vi "Read Name.vi"(8 "error in (no error)":errorcluster, 11 "Process In":refnum<class "Process.lvclass">) -> (0 "error out":errorcluster, 1 "Name":string, 2 "Qualified Name":string, 3 "Process Out":refnum<class "Process.lvclass">)   [LabVIEW 2020, in "Process.lvclass"]
doc: "Returns the name of the object. The Qualified Name is prepended with the name of the owner recursively in the format \"Owner Name::Name\"."
uses:
  Process.lvclass
  C:/git/astemes-triarc-framework/source/Framework/Base/Base.lvclass
  Process.lvclass/Process.ctl
  Base/Base.lvclass/Base.ctl
  <vilib>/Utility/error.llb/Clear Errors.vi
  <vilib>/Utility/error.llb/Error Cluster From Error Code.vi
  Base/Base.lvclass
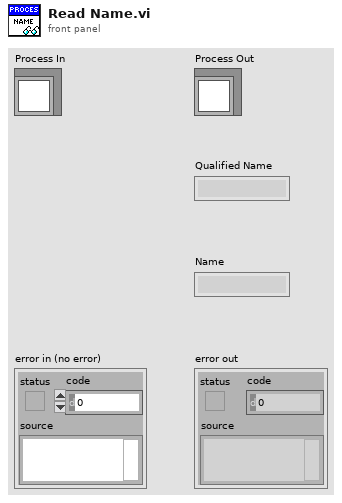
[diagram p1: front panel]
types:
  T1 = typedef "Process.lvclass/Lifecycle State.ctl" = enum16{"Uninitialized", "Initialized", "Started", "Running", "Stopped", "Finished"}
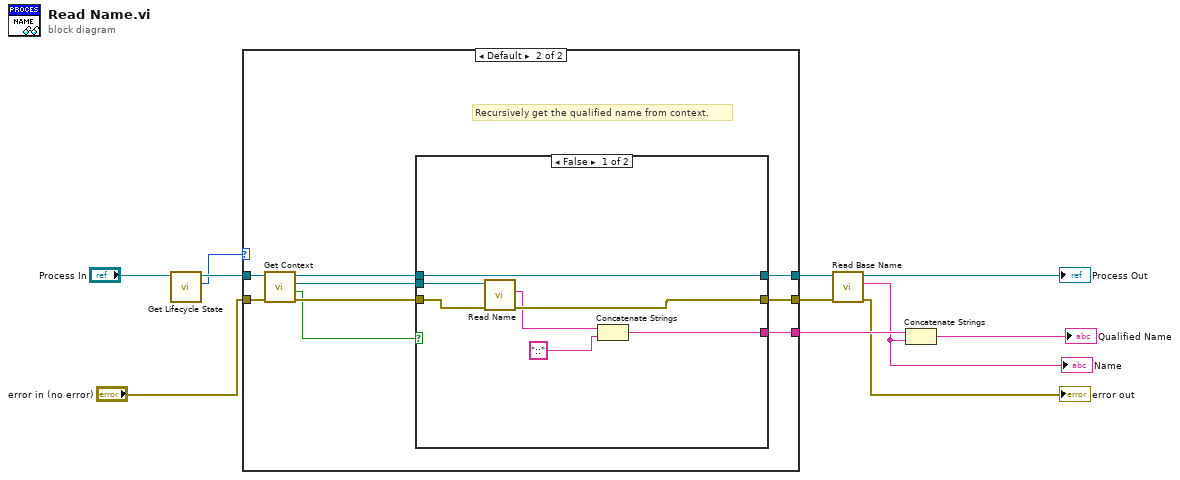
[diagram p0: block diagram]
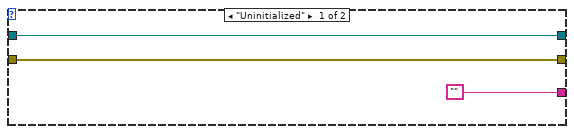
[diagram p2: hidden frame]
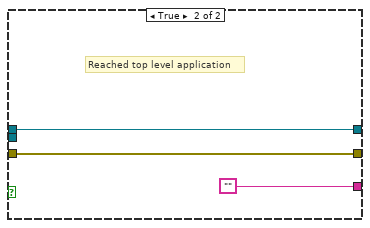
[diagram p3: hidden frame]
diagram:
  n1 = call "Get Lifecycle State.vi"("Process In"="Process In") -> ("Lifecycle State"=w2:T1, "Process Out"=w3:refnum<class "Process.lvclass">)  [unwired: 7 in, 2 out]
  n2 = case shown="Default" w2 {
    tunnel: [w14 w23] -> w10
    tunnel: ["" w22] -> w8
    tunnel: [w13 w21] -> w5
    tunnel: w3 -> [w14 w20]
    tunnel: "error in (no error)" -> [w13 w19]
    frame "Uninitialized" {
    }
    frame Default {
      # "Recursively get the qualified name from context."
      n3 = call "Get Context.vi"("error in (no error)"=w19, "Process In"=w20) -> ("error out"=w16:errorcluster, "Top Level?"=w15:bool, "Context"=w17:refnum<class "Process.lvclass">, "Process Out"=w18:refnum<class "Process.lvclass">)  [unwired: 6 in]
      n4 = case shown="False" w15 {
        tunnel: w17 -> [w30 _]
        tunnel: w18 -> [w29 w33]
        tunnel: [w28 w31] -> w21
        tunnel: [w29 w33] -> w23
        tunnel: [w26 ""] -> w22
        tunnel: w16 -> [w24 w31]
        frame False {
          n5 = call "Read Name.vi"("error in (no error)"=w24, "Process In"=w30) -> ("error out"=w28:errorcluster, "Qualified Name"=w25:string)  [unwired: 6 in, 2 out]
          n6 = Concatenate Strings(w25, "::" ("delimiter")) -> (w26:string)
        }
        frame True {
          # "Reached top level application"
        }
      }
    }
  }
  n7 = call "Read Base Name.vi"("error in (no error)"=w5, "Base In"=w10) -> ("error out"=→"error out":errorcluster, "Name"=w7:string, "Base Out"=→"Process Out":refnum<class "Process.lvclass">)  [unwired: 7 in]
  "Name" <- w7
  n8 = Concatenate Strings(w8, w7) -> (→"Qualified Name":string)
